vi "Read All Sessions Keys and Values.vi"(8 "error in (no error)":errorcluster, 11 "appended path":path) -> (0 "error out":errorcluster, 3 "Device Settings":T1[](array[typedef]))   [LabVIEW 2021]
uses:
  TypeDefs/Device Settings.ctl
  <vilib>/Utility/config.llb/Read Key (String).vi
  <vilib>/Utility/config.llb/NI_LVConfig.lvlib
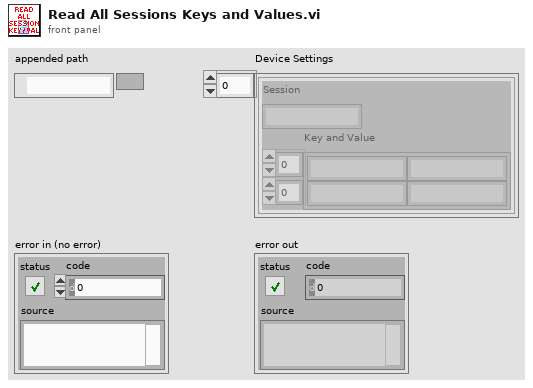
[diagram p1: front panel]
types:
  T1 = typedef "Device Settings.ctl" = cluster{"Session":string, "Key and Value":string[][]}
  T2 = typedef "NI_LVConfig.lvlib/Config Data RefNum.ctl" = refnum<k1>
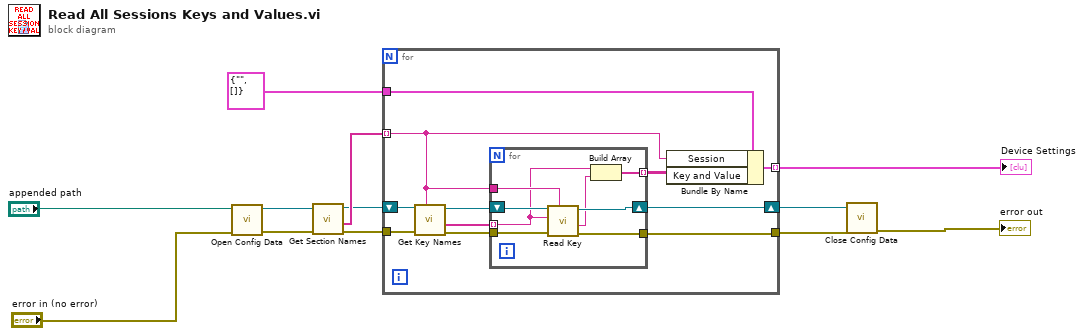
[diagram p0: block diagram]
diagram:
  n1 = call <vilib>:"Open Config Data.vi"("error in (no error)"="error in (no error)", "configuration file path"="appended path") -> ("error out"=w3:errorcluster, "refnum"=w2:T2)  [unwired: 7 in, 1 out]
  n2 = call <vilib>:"Get Section Names.vi"("error in (no error)"=w3, "refnum"=w2) -> ("error out"=w6:errorcluster, "section names"=w7:string[], "refnum out"=w5:T2)  [unwired: 7 in]
  n3 = for {
    tunnel: w6 -> [w22]
    tunnel: w7 -> [w16] mode=indexing
    shift-right: [w18] -> w9
    shift-left: w5 -> [w23]
    tunnel: [w15] -> w8 mode=indexing
    tunnel: [w14] -> w10
    tunnel: T1 {"Session"="", "Key and Value"=[]} ("Configure Cluster") -> [w13]
    n4 = call <vilib>:"Get Key Names.vi"("section"=w16, "error in (no error)"=w22, "refnum"=w23) -> ("error out"=w19:errorcluster, "key names"=w21:string[], "refnum out"=w20:T2)  [unwired: 5 in, 1 out]
    n5 = for {
      tunnel: w16 -> [w31]
      tunnel: w21 -> [w27] mode=indexing
      tunnel: w19 -> [w29]
      shift-right: [w28] -> w18
      shift-left: w20 -> [w30]
      tunnel: [w25] -> w17 mode=indexing
      tunnel: [w24] -> w14
      n6 = call-poly <vilib>:"Read Key.vi"("section"=w31, "error in (no error)"=w29, "key"=w27, "refnum"=w30) -> ("error out"=w24:errorcluster, "value"=w26:string, "refnum out"=w28:T2)  [unwired: 4 in, 1 out]
      n7 = Build Array(w27, w26) -> (w25:string[])
    }
    n8 = Bundle By Name(cluster=w13, "Session"=w16, "Key and Value"=w17) -> (w15:T1)
  }
  "Device Settings" <- w8
  n9 = call <vilib>:"Close Config Data.vi"("error in (no error)"=w10, "refnum"=w9) -> ("error out"=→"error out":errorcluster)  [unwired: 8 in, 1 out]
